vi "MenuHandler.vi"(5 "tree control":refnum<vi>, 7 "main queue":refnum<queue>, 8 "error in":errorcluster, 9 "parameters":variant, 10 "menu string":string, 11 "Abstract Engine":refnum<class "Abstract Engine.lvclass">) -> (0 "error out":errorcluster, 1 "refresh tree?":bool, 2 "Unhandled":bool, 3 "Abstract Engine out":refnum<class "Abstract Engine.lvclass">)   [LabVIEW 2025, in "Abstract Engine.lvlib" / "Abstract Engine.lvclass"]
doc: "Copyright 2017 National Instruments Corporation\n\nLicensed under the Apache License, Version 2.0 (the \"License\"); you may not use this file except in compliance with the License. You may obtain a copy of the License at http://www.apache.org/licenses/LICENSE-2.0\nUnless required by applicable law or agreed to in writing, software distributed under the License is distributed on an \"AS IS\" BASIS, WITHOUT WARRANTIES OR CONDITIONS OF ANY KIND, either express or implied. See the License for the specific language governing permissions and limitations under the License."
uses:
  Abstract Engine.lvclass
  Users/Public/Documents/Sandia National Labs/TSS Plugin/CEF.lvlibp/serializable node/CEF_serializable node.lvclass
  Abstract Engine.lvclass/Abstract Engine.ctl
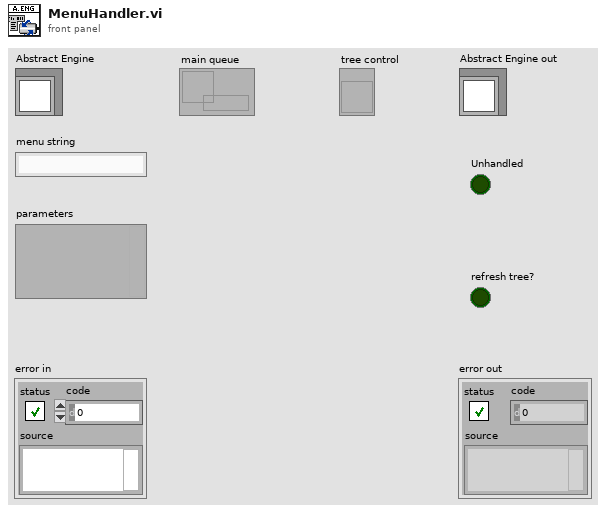
[diagram p1: front panel]
types:
  T1 = cluster{"notification":string, "Engine Data":string[]}
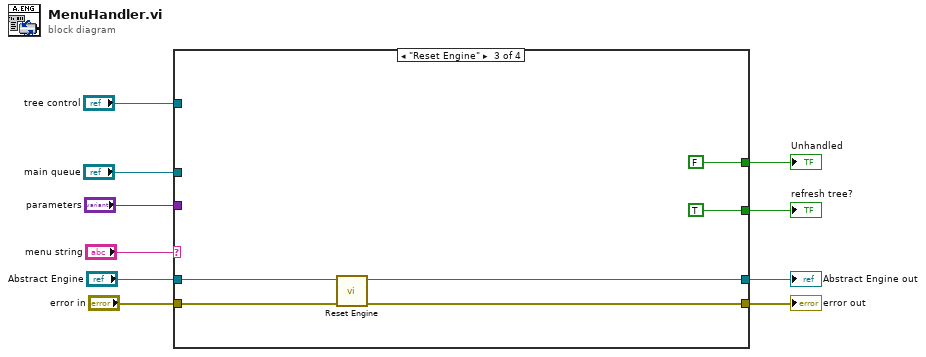
[diagram p0: block diagram]
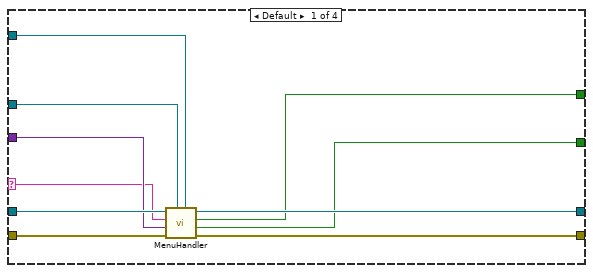
[diagram p2: hidden frame]
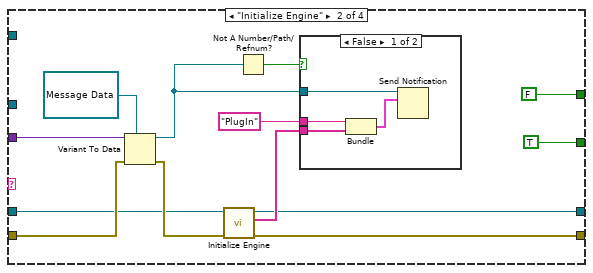
[diagram p3: hidden frame]
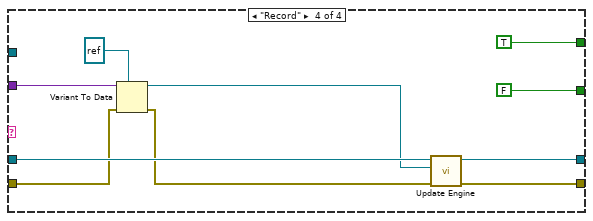
[diagram p5: hidden frame]
diagram:
  n1 = case shown="\"Reset Engine\"" "menu string" {
    selector: "menu string" -> [w15 _ _ _]
    tunnel: "Abstract Engine" -> [w18 w25 w43 w53]
    tunnel: "error in" -> [w20 w29 w41 w46]
    tunnel: [w19 w23 w40 w47] -> w7
    tunnel: [w17 w22 w42 w52] -> w6
    tunnel: [w12 FALSE ("Unhandled") FALSE ("Unhandled") TRUE ("Unhandled")] -> w5
    tunnel: [w11 TRUE ("refresh tree?") TRUE ("refresh tree?") FALSE ("refresh tree?")] -> w4
    tunnel: "parameters" -> [w16 w31 _ w49]
    tunnel: "main queue" -> [w14 _ _ _]
    tunnel: "tree control" -> [w13 _ _ _]
    frame Default {
      n2 = call-parent "MenuHandler.vi"("tree control"=w13, "main queue"=w14, "error in"=w20, "parameters"=w16, "menu string"=w15, "CEF_serializable node in"=w18) -> ("error out"=w19:errorcluster, "refresh tree?"=w11:bool, "Unhandled"=w12:bool, "CEF_serializable node out"=w17:refnum<class "Abstract Engine.lvclass">)  [unwired: 2 in]
    }
    frame "Initialize Engine" {
      n3 = Variant To Data(error in=w29, type=refnum<notifier> refnum ("notifier"), Variant=w31) -> (data=w27:refnum<notifier>, error out=w26:errorcluster)
      n4 = call "Initialize Engine.vi"("error in (no error)"=w26, "Abstract Engine"=w25) -> ("error out"=w23:errorcluster, "Engine Data"=w24:string[], "Abstract Engine out"=w22:refnum<class "Abstract Engine.lvclass">)  [unwired: 7 in]
      n5 = Not A Number/Path/Refnum?(number/path/refnum=w27) -> (NaN/Path/Refnum?=w28:bool)
      n6 = case shown="False" w28 {
        tunnel: w27 -> [w37 _]
        tunnel: w24 -> [w35 _]
        tunnel: "PlugIn" ("notification") -> [w34 _]
        frame False {
          n7 = Bundle("notification"=w34, "Engine Data"=w35) -> (w36:T1)  [unwired: 1 in]
          n8 = Send Notification(notification=w36, notifier=w37) -> ()  [unwired: 1 in, 2 out]
        }
        frame True {
        }
      }
    }
    frame "Reset Engine" {
      n9 = call "Reset Engine.vi"("error in (no error)"=w41, "Abstract Engine"=w43) -> ("error out"=w40:errorcluster, "Abstract Engine out"=w42:refnum<class "Abstract Engine.lvclass">)  [unwired: 8 in]
    }
    frame "Record" {
      n10 = Variant To Data(error in=w46, type=refnum<k34> refnum ("tdms file"), Variant=w49) -> (data=w48:refnum<k34>, error out=w45:errorcluster)
      n11 = call "Update Engine.vi"("error in (no error)"=w45, "tdms ref"=w48, "Abstract Engine"=w53) -> ("error out"=w47:errorcluster, "Abstract Engine out"=w52:refnum<class "Abstract Engine.lvclass">)  [unwired: 7 in]
    }
  }
  "error out" <- w7
  "Abstract Engine out" <- w6
  "Unhandled" <- w5
  "refresh tree?" <- w4
